vi "Host_Init.vi"(9 "Lot No":string, 10 "Recipe Name":string, 11 "Recipe Dir":path) -> (0 "error out":errorcluster, 1 "Camera":refnum<k5>, 2 "Motion":refnum<visa-resource-name>, 3 "Recipe":T1, 6 "MES OK":bool, 7 "MES Code":string)   [LabVIEW 2018]
doc: "Use this template to build a VI to use as a subVI."
uses:
  reuse/10 MES Folder-2/08_Alarm/Recipe.ctl
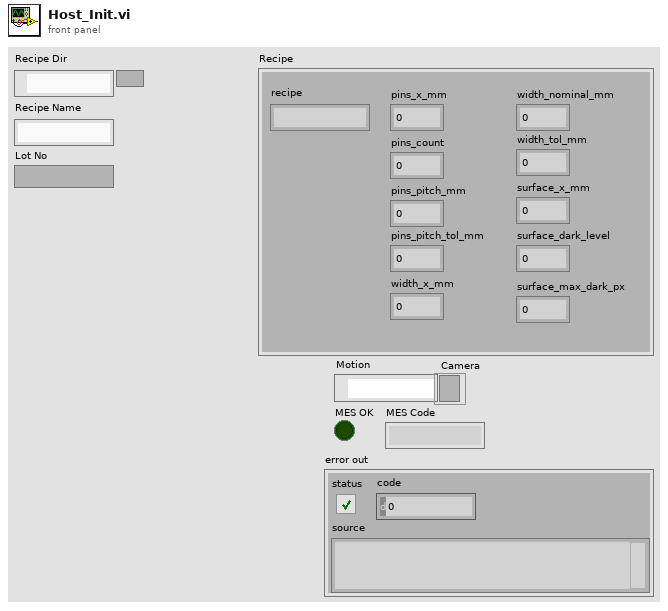
[diagram p1: front panel]
types:
  T1 = typedef "Recipe.ctl" = cluster{"recipe":string, "pins_x_mm":dbl, "pins_count":i32, "pins_pitch_mm":dbl, "width_x_mm":dbl, "width_nominal_mm":dbl, "surface_max_dark_px":i32, "surface_dark_level":dbl, "surface_x_mm":dbl, "width_tol_mm":dbl, "pins_pitch_tol_mm":dbl}
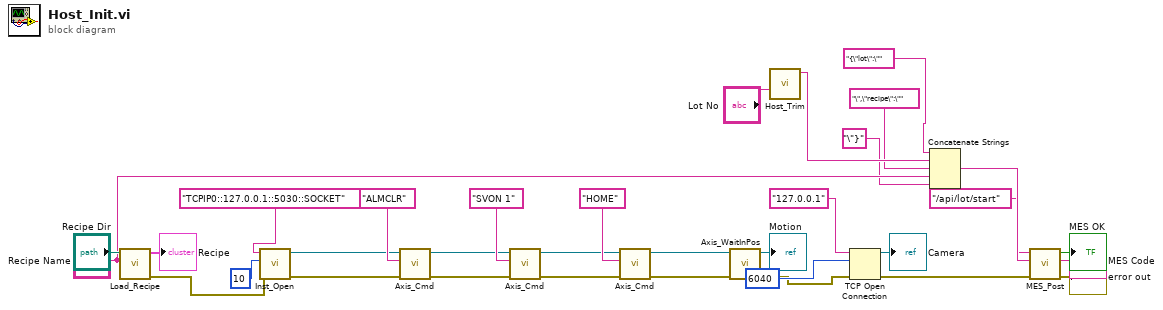
[diagram p0: block diagram]
diagram:
  n1 = call "Load_Recipe.vi"("Recipe Name"="Recipe Name", "Recipe Dir"="Recipe Dir") -> ("error out"=w28:errorcluster, "Recipe"=→"Recipe":T1)  [unwired: 8 in]
  n2 = call "Inst_Open.vi"("error in (no error)"=w28, "TermChar"=u8 10, "VISA Refnum in"="TCPIP0::127.0.0.1::5030::SOCKET") -> ("error out"=w25:errorcluster, "VISA Refnum out"=w26:refnum<visa-resource-name>)  [unwired: 7 in]
  n3 = call "Axis_Cmd.vi"("error in (no error)"=w25, "Command"="ALMCLR", "VISA Refnum name"=w26) -> ("error out"=w22:errorcluster, "VISA Refnum name out"=w23:refnum<visa-resource-name>)  [unwired: 6 in, 1 out]
  n4 = call "Axis_Cmd.vi"("error in (no error)"=w22, "Command"="SVON 1", "VISA Refnum name"=w23) -> ("error out"=w19:errorcluster, "VISA Refnum name out"=w20:refnum<visa-resource-name>)  [unwired: 6 in, 1 out]
  n5 = call "Axis_Cmd.vi"("error in (no error)"=w19, "Command"="HOME", "VISA Refnum name"=w20) -> ("error out"=w17:errorcluster, "VISA Refnum name out"=w18:refnum<visa-resource-name>)  [unwired: 6 in, 1 out]
  n6 = call "Axis_WaitInPos.vi"("error in (no error)"=w17, "VISA Refnum name"=w18) -> ("error out"=w13:errorcluster, "visa out"=→"Motion":refnum<visa-resource-name>)  [unwired: 8 in]
  n7 = call "Host_Trim.vi"("string"="Lot No") -> ("trimmed string"=w9:string)  [unwired: 10 in]
  n8 = TCP Open Connection(address="127.0.0.1", remote port or service name=u16 6040, error in (no error)=w13) -> (connection ID=→"Camera":refnum<k5>, error out=w4:errorcluster)  [unwired: 2 in]
  n9 = Concatenate Strings("{\"lot\":\"", w9, "\",\"recipe\":\"", "Recipe Name", "\"}") -> (w6:string)
  n10 = call "MES_Post.vi"("error in (no error)"=w4, "Body"=w6, "Path"="/api/lot/start") -> ("error out"=→"error out":errorcluster, "Code"=→"MES Code":string, "MES OK"=→"MES OK":bool)  [unwired: 5 in, 1 out]
